vi "RemoteVI Read Client Bytes.vi"(0 "connection":u32, 5 "rx buffer":string) -> (4 "rx buffer out":string, 6 "gone?":bool)   [LabVIEW 2020, in "RemoteVI.lvlib"]
doc: "Reads whatever bytes a WebSocket client has sent WITHOUT waiting (TCP Read, immediate mode, timeout 0, 64 KiB at most) and appends them to rx buffer. gone? is TRUE when the read reported any error other than 56 (timeout - nothing waiting), i.e. the peer closed or reset the connection. connection is the TCP connection refnum type-cast to U32."
uses:
  RemoteVI.lvlib
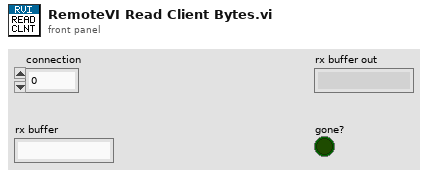
[diagram p1: front panel]
types:
  T1 = enum16{"standard", "buffered", "CRLF", "immediate"}
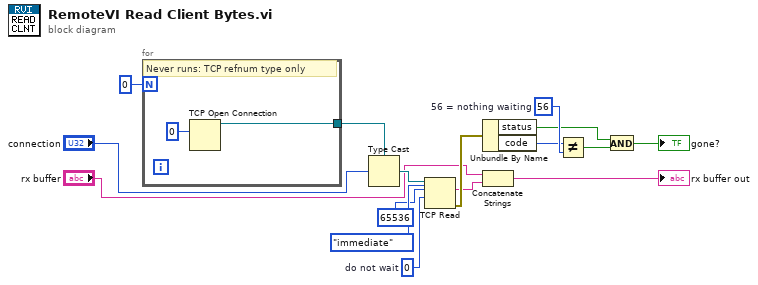
[diagram p0: block diagram]
diagram:
  w14 = 56  # 56 = nothing waiting
  w7 = 0  # do not wait
  n1 = for {
    N: 0 -> [_]
    tunnel: [w18] -> w4
    # "Never runs: TCP refnum type only"
    n2 = TCP Open Connection(remote port or service name=u16 0) -> (connection ID=w18:refnum<k5>)  [unwired: 4 in, 1 out]
  }
  n3 = Type Cast(type=w4, x="connection") -> (*(type *) &x=w5:refnum<k5>)
  n4 = TCP Read(connection ID=w5, bytes to read=65536, 7:T1."immediate", 9:w7) -> (data out=w9:string, error out=w10:errorcluster)  [unwired: 1 in, 1 out]
  n5 = Unbundle By Name(w10) -> ("status"=w12:bool, "code"=w13:i32)
  n6 = Concatenate Strings("rx buffer", w9) -> (→"rx buffer out":string)
  n7 = Not Equal?(x=w13, y=w14) -> (x != y?=w15:bool)
  n8 = And(x=w12, y=w15) -> (x .and. y?=→"gone?":bool)
